vi "set Detector Mode.vi"(6 "Detect Auto?":bool, 8 "error in (no error)":errorcluster, 9 "Trace Index":u32=1 min=1, 10 "Detector Type":T1=enum."Auto Peak", 11 "FSV-40N in":refnum<class "FSV-40N.lvclass">) -> (0 "error out":errorcluster, 3 "FSV-40N out":refnum<class "FSV-40N.lvclass">)   [LabVIEW 2023, in "Spectrum Analyzer.lvlib" / "FSV-40N.lvclass"]
uses:
  FSV-40N.lvclass
  TYPE DEFINITION/TYPE Detect Mode Select.ctl
  FSV-40N.lvclass/FSV-40N.ctl
  Spectrum Analyzer.lvlib
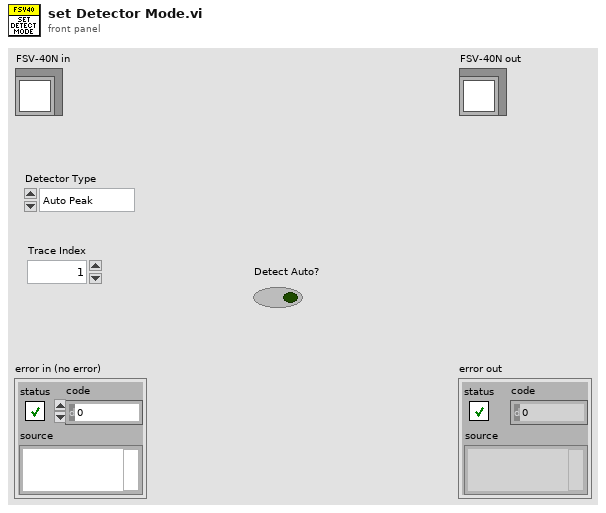
[diagram p1: front panel]
types:
  T1 = typedef "Spectrum Analyzer.lvlib/TYPE Detect Mode Select.ctl" = enum16{"Det Auto", "Auto Peak", "Positive Peak", "Negative Peak", "Sample", "RMS", "Average", "Quasipeak", "CISPR Average", "RMS Average"}
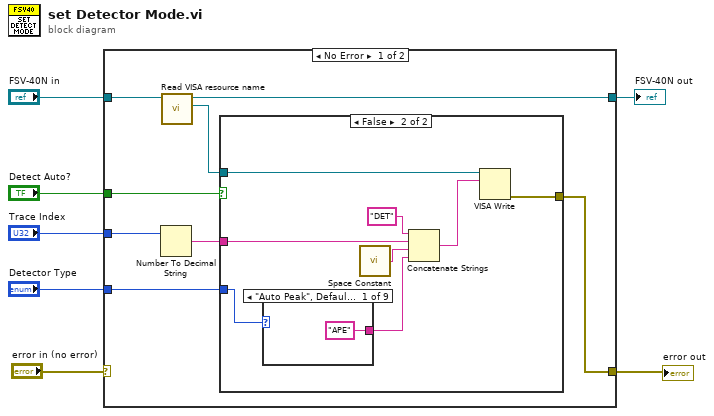
[diagram p0: block diagram]
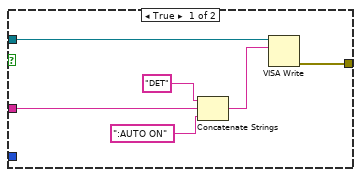
[diagram p2: hidden frame]
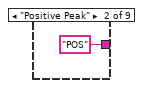
[diagram p3: hidden frame]
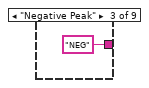
[diagram p4: hidden frame]
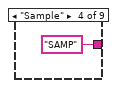
[diagram p5: hidden frame]
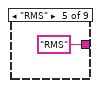
[diagram p6: hidden frame]
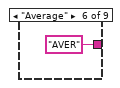
[diagram p7: hidden frame]
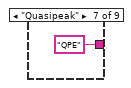
[diagram p8: hidden frame]
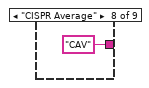
[diagram p9: hidden frame]
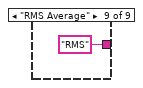
[diagram p10: hidden frame]
diagram:
  n1 = case shown="No Error" "error in (no error)" {
    selector: "error in (no error)" -> [_ w39]
    tunnel: "FSV-40N in" -> [w15 w40]
    tunnel: [w8 w40] -> w5
    tunnel: [w9 w39] -> w4
    tunnel: "Detect Auto?" -> [w13 _]
    tunnel: "Trace Index" -> [w12 _]
    tunnel: "Detector Type" -> [w10 _]
    frame No Error {
      n2 = Number To Decimal String(number=w12) -> (decimal integer string=w11:string)  [unwired: 1 in]
      n3 = call "Read VISA resource name.vi"("FSV-40N in"=w15) -> ("VISA resource name"=w14:refnum<visa-resource-name>, "FSV-40N out"=w8:refnum<class "FSV-40N.lvclass">)  [unwired: 8 in, 1 out]
      n4 = case shown="False" w13 {
        tunnel: w14 -> [w21 w29]
        tunnel: w11 -> [w20 w28]
        tunnel: [w16 w25] -> w9
        tunnel: w10 -> [_ w24]
        frame True {
          n5 = Concatenate Strings("DET" ("string"), w20, ":AUTO ON" ("string")) -> (w17:string)
          n6 = VISA Write(VISA resource name=w21, write buffer=w17) -> (error out=w16:errorcluster)  [unwired: 1 in, 2 out]
        }
        frame False {
          n7 = case shown="\"Auto Peak\", Default" w24 {
            tunnel: ["APE" ("string") "POS" ("string") "NEG" ("string") "SAMP" ("string") "RMS" ("string") "AVER" ("string") "QPE" ("string") "CAV" ("string") "RMS" ("string")] -> w22
            frame "Auto Peak", Default {
            }
            frame "Positive Peak" {
            }
            frame "Negative Peak" {
            }
            frame "Sample" {
            }
            frame "RMS" {
            }
            frame "Average" {
            }
            frame "Quasipeak" {
            }
            frame "CISPR Average" {
            }
            frame "RMS Average" {
            }
          }
          n8 = call <vilib>:"Space Constant.vi"() -> ("String"=w23:string)
          n9 = Concatenate Strings("DET" ("string"), w28, w23, w22) -> (w26:string)
          n10 = VISA Write(VISA resource name=w29, write buffer=w26) -> (error out=w25:errorcluster)  [unwired: 1 in, 2 out]
        }
      }
    }
    frame Error {
    }
  }
  "error out" <- w4
  "FSV-40N out" <- w5
